vi "base array selection data read.vi"(8 "error in":errorcluster, 9 "stripped path":path, 10 "selection":i32, 11 "filenames":string[](array[string])) -> (0 "error out":errorcluster, 2 "element":string, 3 "Base All Composition":T1(array[cluster]))   [LabVIEW 2018]
panel:
  out "Base Species IDX":i32
  out "ex":string
  out "Base Color":u32
  out "R Base Level":dbl
  out "R STD Level":dbl
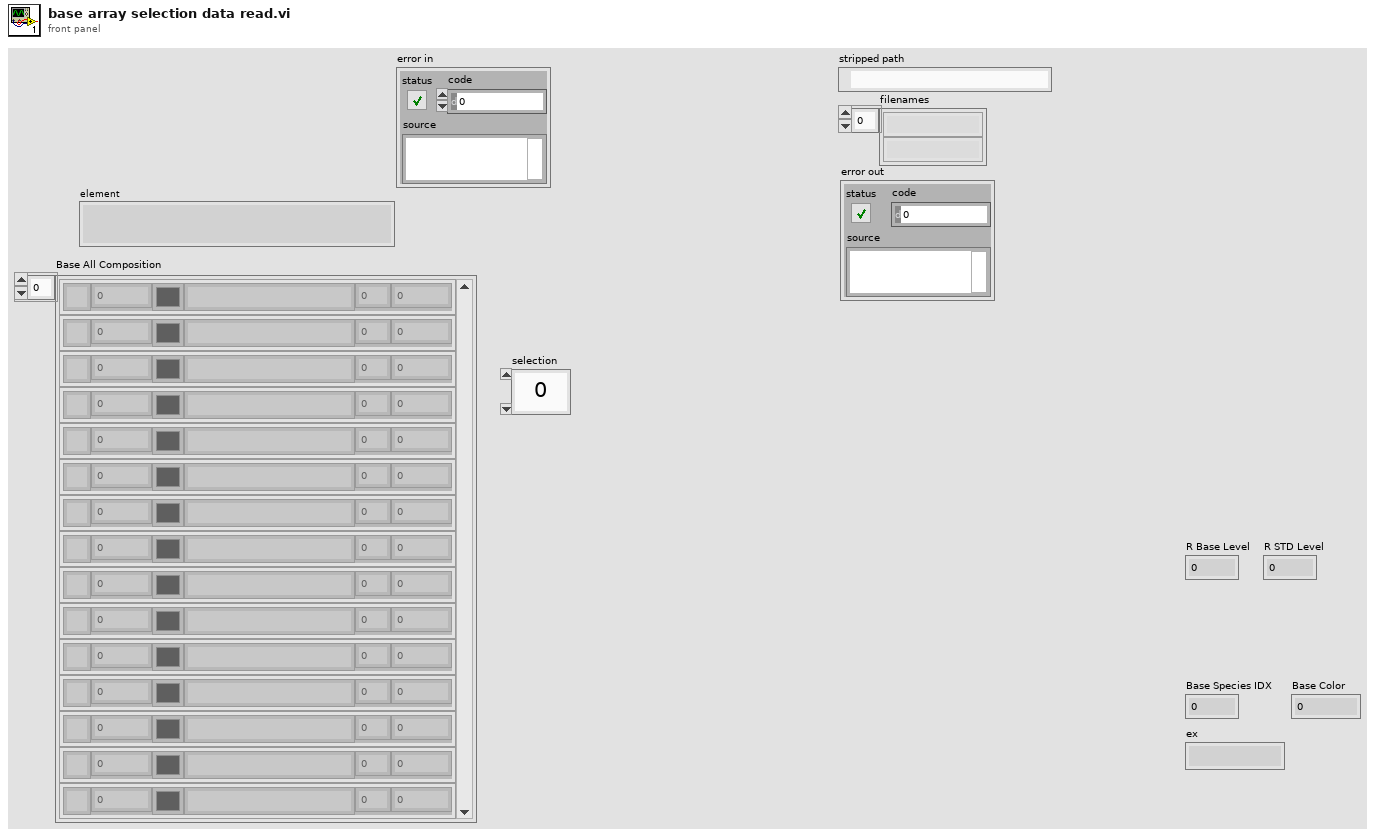
[diagram p1: front panel]
types:
  T1 = cluster{"Name":string, "Value":dbl, "Color":u32, "Name 2":string, "Value 2":dbl, "Value 3":dbl}[]
  T2 = cluster{"String":string, dbl, i32, "String":string, i32, dbl}[]
  T3 = cluster{"String":string, dbl, i32, "String":string, i32, dbl}
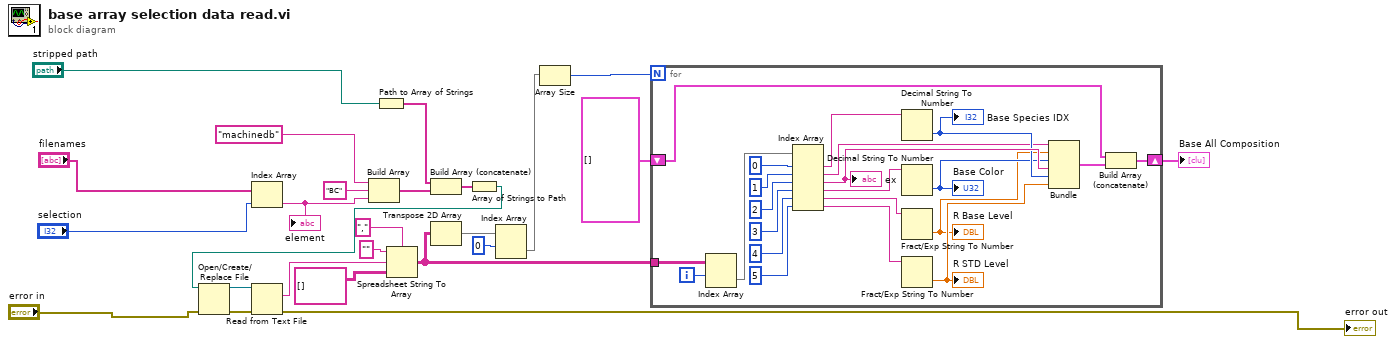
[diagram p0: block diagram]
diagram:
  n1 = Index Array(array="filenames", index="selection") -> (element=w22:string)
  "element" <- w22
  n2 = Build Array("machinedb", "BC", w22) -> (w20:string[])
  n3 = Path to Array of Strings(0:"stripped path") -> (2:w21:string[])  [unwired: 1 out]
  n4 = Build Array (concatenate)(w21, w20) -> (w19:string[])
  n5 = Array of Strings to Path(0:w19) -> (2:w5:path)  [unwired: 1 in]
  n6 = Open/Create/Replace File(file path (use dialog)=w5, error in="error in") -> (refnum out=w12:refnum<file>, error out=w11:errorcluster)  [unwired: 4 in, 1 out]
  n7 = Read from Text File(file (use dialog)=w12, error in=w11) -> (text=w13:string, error out=→"error out":errorcluster)  [unwired: 2 in, 2 out]
  n8 = Spreadsheet String To Array(delimiter (Tab)=",", format string="", spreadsheet string=w13, array type (2D Dbl)=string[][] []) -> (array=w14:string[][])
  n9 = Transpose 2D Array(2D array=w14) -> (transposed array=w18:string[][])
  n10 = Index Array(array=w18, index (row)=0 ("index")) -> (element=w15:string[])  [unwired: 1 in]
  n11 = Array Size(array=w15) -> (size(s)=w16:i32)
  n12 = for {
    N: w16 -> [_]
    tunnel: w14 -> [w30]
    shift-right: [w26] -> w17
    shift-left: T2 [] -> [w28]
    i -> [w29]
    n13 = Index Array(array=w30, index (row)=w29) -> (element=w37:string[])  [unwired: 1 in]
    n14 = Index Array(array=w37, index #1=0 ("index"), index #2=1 ("index"), index #3=2 ("index"), index #4=3 ("index"), index #5=4 ("index"), index #6=5 ("index")) -> (element #1=w38:string, element #2=w39:string, element #3=w47:string, element #4=w42:string, element #5=w40:string, element #6=w44:string)
    "ex" <- w47
    n15 = Decimal String To Number(string=w38) -> (number=w45:i32)  [unwired: 2 in, 1 out]
    "Base Species IDX" <- w45
    n16 = Decimal String To Number(string=w42) -> (number=w43:i32)  [unwired: 2 in, 1 out]
    "Base Color" <- w43
    n17 = Fract/Exp String To Number(string=w40) -> (number=w41:dbl)  [unwired: 3 in, 1 out]
    "R Base Level" <- w41
    n18 = Fract/Exp String To Number(string=w44) -> (number=w46:dbl)  [unwired: 3 in, 1 out]
    "R STD Level" <- w46
    n19 = Bundle("String"=w39, w41, w43, "String"=w47, w45, w46) -> (w27:T3)  [unwired: 1 in]
    n20 = Build Array (concatenate)(w28, w27) -> (w26:T2)
  }
  "Base All Composition" <- w17
